vi "Add USB Relay Error.vi"(8 "error in (no error)":errorcluster, 9 "String to Append":string, 10 "Error":T1, 11 "Insert Error":bool=TRUE) -> (0 "error out":errorcluster)   [LabVIEW 2021, in "USB Relay Control.lvlib"]
doc: "This VI will insert a custome error message. This wrapper is designed to be inlined to minimize overhead when there is no error. It calls an error core VI that should not be inlined to minimize memory impact."
uses:
  USB Relay Control.lvlib
  typedef/Errors.ctl
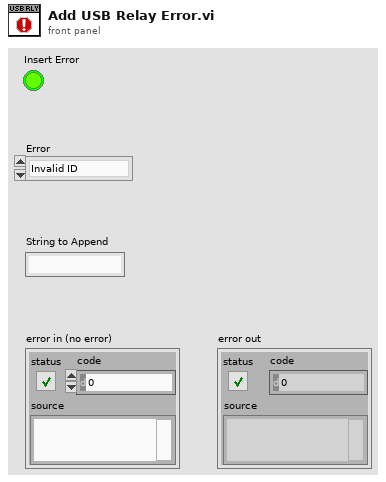
[diagram p1: front panel]
types:
  T1 = typedef "USB Relay Control.lvlib/Errors.ctl" = enum16{"Invalid ID"}
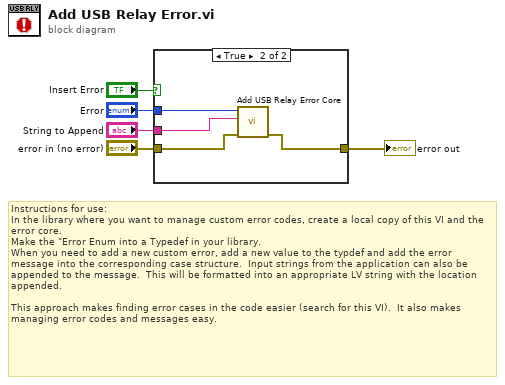
[diagram p0: block diagram]
diagram:
  # "Instructions for use:\nIn the library where you want to manage custom error codes, create a local copy of this VI and the error core.\nMake the \"Error Enum into a Typedef in your library.\nWhen you need to add a new custom error, add a new value to the typdef and add the error message into the corresponding case structure.  Input strings from the application can also be appended to the message.  This will be formatted into an appropriate LV string with the location appended.  \n\nThis approach makes finding error cases in the code easier (search for this VI).  It also makes managing error codes and messages easy."
  n1 = case shown="True" "Insert Error" {
    tunnel: [w6 w7] -> w4
    tunnel: "error in (no error)" -> [w6 w8]
    tunnel: "Error" -> [_ w10]
    tunnel: "String to Append" -> [_ w9]
    frame False {
    }
    frame True {
      n2 = call "Add USB Relay Error Core.vi"("error in (no error)"=w8, "String to Append"=w9, "Error"=w10) -> ("error out"=w7:errorcluster)  [unwired: 8 in]
    }
  }
  "error out" <- w4
